vi "onUnsubscribe.vi"(6 "timeout (1000ms)":i32=1000, 8 "error in (no error)":errorcluster, 10 "UNSUBSCRIBE":refnum<class "UNSUBSCRIBE.lvclass">, 11 "Client in":refnum<class "Client.lvclass">) -> (0 "error out":errorcluster, 1 "Ack":bool, 2 "UNSUBACK":refnum<class "UNSUBACK.lvclass">, 3 "Client out":refnum<class "Client.lvclass">)   [LabVIEW 2013, in "MQTT Client.lvlib" / "Client.lvclass"]
uses:
  Client.lvclass
  <vilib>/LabVIEW Open Source Project/MQTT Control Packets/Control Packets/UNSUBSCRIBE/UNSUBSCRIBE.lvclass
  <vilib>/LabVIEW Open Source Project/MQTT Control Packets/Control Packets/UNSUBACK/UNSUBACK.lvclass
  <vilib>/LabVIEW Open Source Project/MQTT Control Packets/Control Packets/ControlPacket/ControlPacket.lvclass/ControlPacket.ctl
  Session.Client/Session.Client.lvclass
  <vilib>/LabVIEW Open Source Project/MQTT Control Packets/Control Packets/ControlPacket/ControlPacket.lvclass
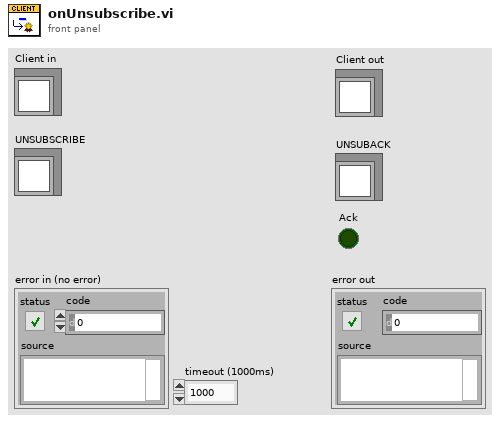
[diagram p1: front panel]
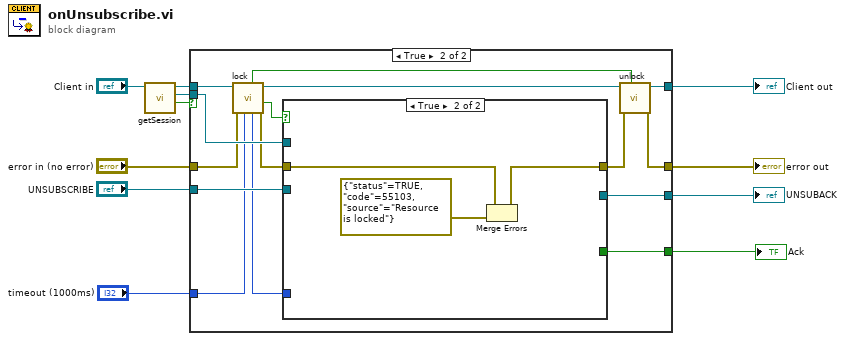
[diagram p0: block diagram]
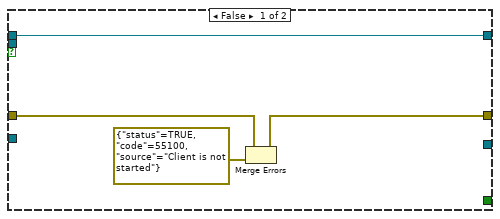
[diagram p2: hidden frame]
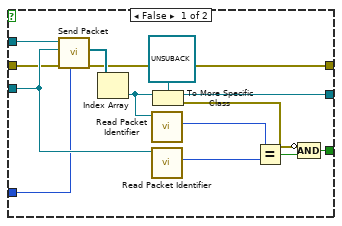
[diagram p3: hidden frame]
diagram:
  n1 = call "getSession.vi"("Client in"="Client in") -> ("valid?"=w7:bool, "Session"=w8:refnum<class "Session.Client.lvclass">, "Client out"=w6:refnum<class "Client.lvclass">)  [unwired: 8 in]
  n2 = case shown="True" w7 {
    tunnel: "timeout (1000ms)" -> [_ w23]
    tunnel: "UNSUBSCRIBE" -> [_ w30]
    tunnel: [_ w29] -> w10
    tunnel: [_ w28] -> w9
    tunnel: "error in (no error)" -> [w13 w25]
    tunnel: [w12 w18] -> w1
    tunnel: w8 -> [_ w27]
    tunnel: w6 -> [w15 w26]
    tunnel: [w15 w20] -> w2
    frame False {
      n3 = Merge Errors(w13, errorcluster {"status"=TRUE, "code"=55100, "source"="Client is not started"} ("error in")) -> (w12:errorcluster)
    }
    frame True {
      n4 = call "lock.vi"("timeout (2000ms)"=w23, "error in (no error)"=w25, "Client in"=w26) -> ("error out"=w24:errorcluster, "timed out"=w16:bool, "Client out"=w21:refnum<class "Client.lvclass">, "remaining (ms)"=w22:i32, "locked"=w17:bool)  [unwired: 4 in]
      n5 = case shown="True" w16 {
        tunnel: w30 -> [w42 _]
        tunnel: [w41 _] -> w29
        tunnel: [w37 _] -> w28
        tunnel: w27 -> [w36 _]
        tunnel: w24 -> [w33 w46]
        tunnel: w22 -> [w32 _]
        tunnel: [w31 w45] -> w19
        frame False {
          n6 = call "Send Packet.vi"("timeout (0ms : no ack)"=w32, "error in (no error)"=w33, "Packet"=w42, "Session"=w36) -> ("error out"=w31:errorcluster, "Response"=w44:refnum<class "ControlPacket.lvclass">[])  [unwired: 4 in, 2 out]
          n7 = Index Array(array=w44) -> (element=w34:refnum<class "ControlPacket.lvclass">)  [unwired: 1 in]
          n8 = call <vilib>:"Read Packet Identifier.vi"("ControlPacket in"=w34) -> ("Packet Identifier"=w39:u16)  [unwired: 9 in, 1 out]
          n9 = call <vilib>:"Read Packet Identifier.vi"("ControlPacket in"=w42) -> ("Packet Identifier"=w40:u16)  [unwired: 9 in, 1 out]
          n10 = To More Specific Class(target class=refnum<class "UNSUBACK.lvclass"> refnum ("UNSUBACK"), reference=w34) -> (specific class reference=w41:refnum<class "UNSUBACK.lvclass">, error out=w38:errorcluster)  [unwired: 1 in]
          n11 = Equal?(x=w39, y=w40) -> (x = y?=w35:bool)
          n12 = Compound Arithmetic op=AND(invert w38, w35) -> (w37:bool)
        }
        frame True {
          n13 = Merge Errors(w46, errorcluster {"status"=TRUE, "code"=55103, "source"="Resource is locked"} ("error in")) -> (w45:errorcluster)
        }
      }
      n14 = call "unlock.vi"("Unlock?"=w17, "error in (no error)"=w19, "Client in"=w21) -> ("error out"=w18:errorcluster, "Client out"=w20:refnum<class "Client.lvclass">)  [unwired: 7 in]
    }
  }
  "error out" <- w1
  "Client out" <- w2
  "UNSUBACK" <- w10
  "Ack" <- w9
